vi "InitFromXML.vi"(8 "error in (no error)":errorcluster, 10 "XML":string, 11 "Feed_link in":refnum<class "Feed_link.lvclass">) -> (0 "error out":errorcluster, 3 "Feed_link out":refnum<class "Feed_link.lvclass">)   [LabVIEW 2023, in "GettingStartedWindow.lvlib" / "Feed_link.lvclass"]
uses:
  <resource>/modes/FRC/Classes/Feed_link/Feed_link.lvclass
  home/systemcore/natinst/lvaddons/wpilib/1/resource/modes/FRC/Classes/Link/Link.lvclass
  home/systemcore/natinst/lvaddons/wpilib/1/resource/modes/FRC/Classes/ClickableText/ClickableText.lvclass
  <resource>/modes/FRC/Classes/Feed_link/FeedDB_operation.ctl
  <resource>/modes/FRC/Classes/Feed_link/Feed_link.lvclass/Feed_link.ctl
  <resource>/dialog/lvconfig.llb/LV Config Read Boolean.vi
  <resource>/modes/FRC/Classes/ClickableText/ClickableText.lvclass
  <vilib>/NI_RSS/Feed/Feed.lvclass
  <resource>/modes/FRC/Classes/Link/Link.lvclass
  <resource>/modes/FRC/GettingStartedWindow.lvlib
panel:
  in  "format string":string="%s (%d)"
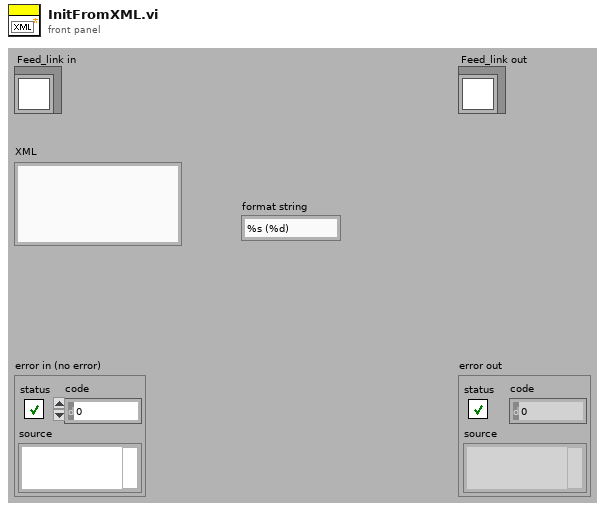
[diagram p1: front panel]
types:
  T1 = typedef "GettingStartedWindow.lvlib/Feed_link.lvclass/FeedDB_operation.ctl" = enum16{"Read All", "Append GUID"}
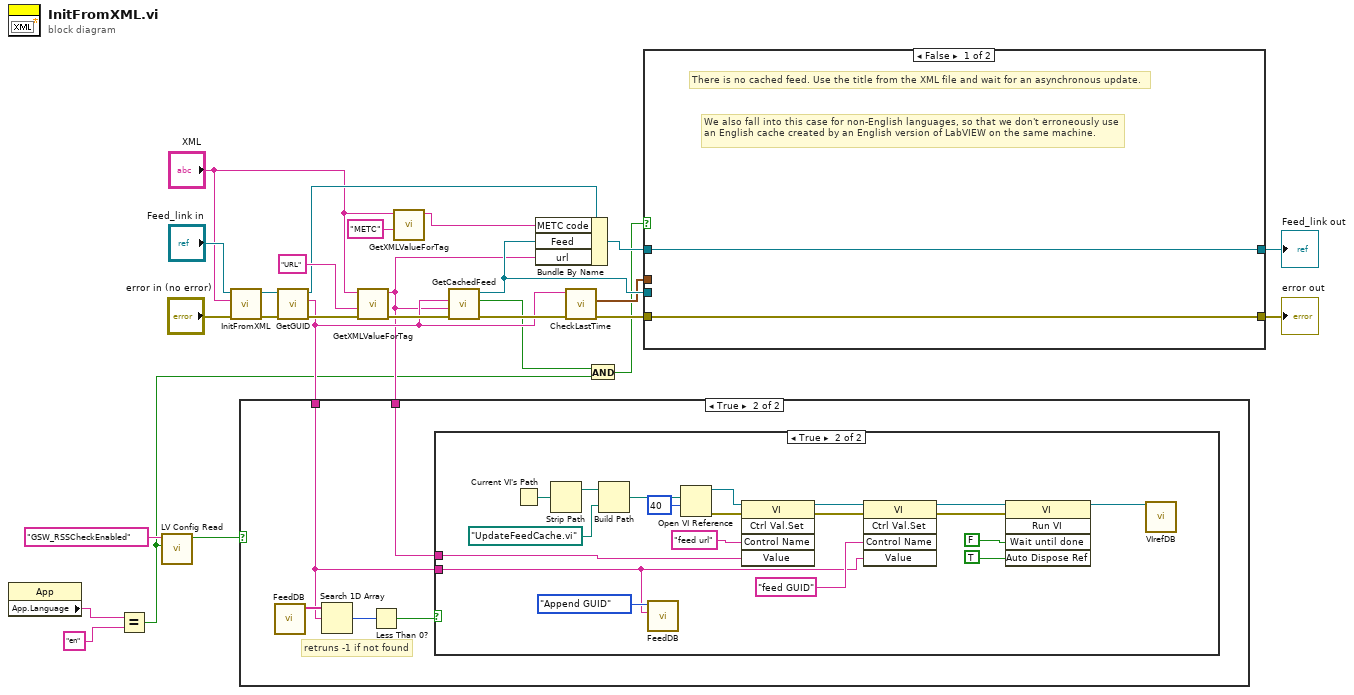
[diagram p0: block diagram]
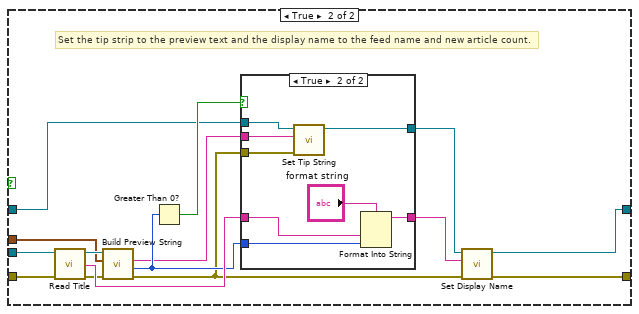
[diagram p4: hidden frame]
diagram:
  n1 = property class="App"() -> ("App.Language"=w5:string)  [unwired: 2 in, 2 out]
  n2 = Equal?(x=w5, y="en") -> (x = y?=w2:bool)
  n3 = call-poly <resource>:"LV Config Read.vi"("default value"=w2, "key"="GSW_RSSCheckEnabled") -> ("value"=w10:bool)  [unwired: 1 in, 4 out]
  n4 = call-parent "InitFromXML.vi"("error in (no error)"="error in (no error)", "XML"="XML", "ClickableText in"="Feed_link in") -> ("error out"=w26:errorcluster, "ClickableText out"=w27:refnum<class "Feed_link.lvclass">)  [unwired: 7 out]
  n5 = call <resource>:"GetGUID.vi"("error in (no error)"=w26, "Link in"=w27) -> ("error out"=w23:errorcluster, "GUID"=w12:string, "Link out"=w13:refnum<class "Feed_link.lvclass">)  [unwired: 7 out]
  n6 = call <resource>:"GetXMLValueForTag.vi"("error in (no error)"=w23, "tag"="URL", "XML"="XML") -> ("error out"=w20:errorcluster, "value"=w6:string)  [unwired: 7 out]
  n7 = case shown="True" w10 {
    tunnel: w6 -> [_ w32]
    tunnel: w12 -> [_ w28]
    frame False {
      # "User has disabled checking RSS feeds in Tools>>Options, so don't spawn the VIs that update the feed."
    }
    frame True {
      # "retruns -1 if not found"
      n8 = call <resource>:"FeedDB.vi"() -> ("updated feeds (GUIDs)"=w30:string[])  [unwired: 2 in, 9 out]
      n9 = Search 1D Array(1D array=w30, element=w28) -> (index of element=w31:i32)  [unwired: 1 out]
      n10 = Less Than 0?(x=w31) -> (x < 0?=w29:bool)
      n11 = case shown="True" w29 {
        tunnel: w32 -> [_ w41]
        tunnel: w28 -> [_ w34]
        frame False {
          # "feed already updated, nothing to do"
        }
        frame True {
          n12 = Current VI's Path() -> (path=w51:path)
          n13 = Strip Path(path=w51) -> (stripped path=w50:path)  [unwired: 1 out]
          n14 = Build Path(base path=w50, name or relative path=path "UpdateFeedCache.vi") -> (appended path=w48:path)
          n15 = call <resource>:"FeedDB.vi"("feed GUID"=w34, "Enum"=FeedDB_operation."Append GUID") -> ()  [unwired: 10 out]
          n16 = Open VI Reference(vi path=w48, options=40) -> (vi reference=w47:refnum<vi>, error out=w45:errorcluster)  [unwired: 1 in, 3 out]
          n17 = invoke class="VI" method="Ctrl Val.Set"(reference=w47, error in=w45, "Control Name"="feed url", "Value"=w41) -> (reference out=w46:refnum<vi>, error out=w44:errorcluster)  [unwired: 1 in, 3 out]
          n18 = invoke class="VI" method="Ctrl Val.Set"(reference=w46, error in=w44, "Control Name"="feed GUID", "Value"=w34) -> (reference out=w40:refnum<vi>, error out=w39:errorcluster)  [unwired: 1 in, 3 out]
          n19 = invoke class="VI" method="Run VI"(reference=w40, error in=w39, "Wait until done"=FALSE ("Wait Until Done"), "Auto Dispose Ref"=TRUE ("Auto Dispose Reference")) -> (reference out=w33:refnum<vi>)  [unwired: 1 in, 4 out]
          n20 = call <resource>:"VIrefDB.vi"("spawned VI ref"=w33) -> ()  [unwired: 11 out]
        }
      }
    }
  }
  n21 = call <resource>:"GetXMLValueForTag.vi"("tag"="METC", "XML"="XML") -> ("value"=w7:string)  [unwired: 1 in, 8 out]
  n22 = call <resource>:"GetCachedFeed.vi"("error in (no error)"=w20, "default URL"=w6, "feed GUID"=w12) -> ("error out"=w16:errorcluster, "cache found"=w3:bool, "Feed"=w21:refnum<class "Feed.lvclass">)  [unwired: 6 out]
  n23 = Bundle By Name(cluster=w13, "METC code"=w7, "Feed"=w21, "url"=w6) -> (w14:refnum<class "Feed_link.lvclass">)
  n24 = call <resource>:"CheckLastTime.vi"("error in (no error)"=w16, "feed GUID"=w12) -> ("error out"=w15:errorcluster, "Time Stamp"=w17:timestamp)  [unwired: 8 out]
  n25 = And(x=w3, y=w2) -> (x .and. y?=w1:bool)
  n26 = case shown="False" w1 {
    tunnel: w21 -> [_ w68]
    tunnel: [w53 w61] -> w19
    tunnel: [w52 w60] -> w18
    tunnel: w17 -> [_ w59]
    tunnel: w15 -> [w52 w58]
    tunnel: w14 -> [w53 w56]
    frame False {
      # "We also fall into this case for non-English languages, so that we don't erroneously use\nan English cache created by an English version of LabVIEW on the same machine."
      # "There is no cached feed. Use the title from the XML file and wait for an asynchronous update."
    }
    frame True {
      # "Set the tip strip to the preview text and the display name to the feed name and new article count."
      n27 = call-dynamic "Read Title.vi"("error in (no error)"=w58, "Feed.lvclass in"=w68) -> ("error out"=w64:errorcluster, "Title"=w66:string, "Feed.lvclass out"=w65:refnum<class "Feed.lvclass">)  [unwired: 7 out]
      n28 = call <vilib>:"Build Preview String.vi"("error in (no error)"=w64, "last checked time stamp"=w59, "Feed in"=w65) -> ("error out"=w55:errorcluster, "new item count"=w63:i32, "preview string"=w57:string)  [unwired: 6 out]
      n29 = Greater Than 0?(x=w63) -> (x > 0?=w67:bool)
      n30 = case shown="True" w67 {
        tunnel: w66 -> [w70 w77]
        tunnel: w63 -> [_ w76]
        tunnel: [w70 w75] -> w62
        tunnel: w56 -> [w69 w74]
        tunnel: w57 -> [_ w73]
        tunnel: w55 -> [_ w72]
        tunnel: [w69 w71] -> w54
        frame False {
        }
        frame True {
          n31 = call <resource>:"Set Tip String.vi"("error in (no error)"=w72, "tip string"=w73, "ClickableText in"=w74) -> ("ClickableText out"=w71:refnum<class "Feed_link.lvclass">)  [unwired: 8 out]
          n32 = Format Into String(format string="format string", w77, w76) -> (resulting string=w75:string)  [unwired: 2 in, 1 out]
        }
      }
      n33 = call <resource>:"Set Display Name.vi"("error in (no error)"=w55, "localized name"=w62, "ClickableText in"=w54) -> ("error out"=w60:errorcluster, "ClickableText out"=w61:refnum<class "Feed_link.lvclass">)  [unwired: 7 out]
    }
  }
  "error out" <- w18
  "Feed_link out" <- w19
